vi "Generate Trace.vi"(11 "String":string) -> ()   [LabVIEW 2020, in "AF Debug.lvlib"]
uses:
  AF Debug.lvlib
  <vilib>/Utility/SystemLogging/NI_SystemLogging.lvlib
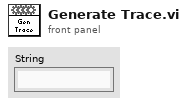
[diagram p1: front panel]
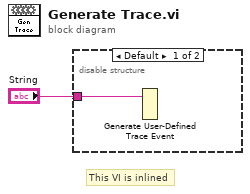
[diagram p0: block diagram]
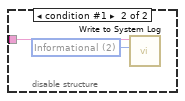
[diagram p2: hidden frame]
diagram:
  # "This VI is inlined"
  n1 = disable-structure shown="Default" {
    disable-tunnel: "String" -> [w2 w4]
    frame condition #0 (active) {
      n2 = Generate User-Defined Trace Event(2:w2) -> ()  [unwired: 1 in]
    }
    frame condition #1 {
      w3 = 2 items=["Error", "Warning", "Informational"] ("severity")
      n3 = call <vilib>:"Write to System Log.vi"("severity"=w3, "message"=w4) -> ()  [unwired: 9 in, 1 out]
    }
  }
